vi "KYFG Scan.vi"(8 "error in (no error)":errorcluster, 10 "count":i32) -> (0 "error out":errorcluster, 2 "infosize":i32, 3 "pids_info":u32[](array[numeric]))   [LabVIEW 2023, in "KYFGLib_lv.lvlib"]
doc: "KYFG_API int KYFG_Scan(unsigned int *pids_info, int count);"
uses:
  KYFGLib_lv.lvlib
  KYFGLib.dll
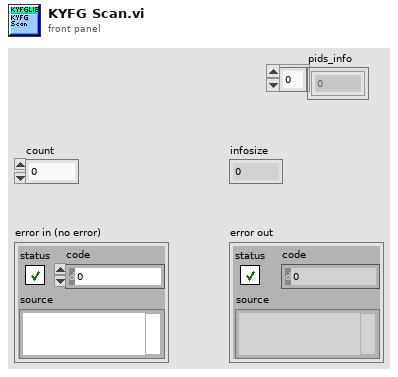
[diagram p1: front panel]
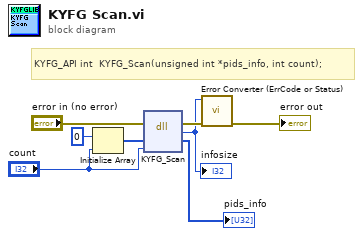
[diagram p0: block diagram]
diagram:
  # "KYFG_API int\t\tKYFG_Scan(unsigned int *pids_info, int count);"
  n1 = Initialize Array(u32 0 ("element"), "count") -> (w1:u32[])
  n2 = dll-call lib="KYFGLib.dll" fn="KYFG_Scan"(error in="error in (no error)", "pids_info"=w1, "count"="count") -> (error out=w7:errorcluster, "return type"=w5:i32, "pids_info"=→"pids_info":u32[])  [unwired: 3 in, 1 out]
  "infosize" <- w5
  n3 = call "Error Converter (ErrCode or Status).vi"("error in (no error)"=w7, "error code"=w5) -> ("error out"=→"error out":errorcluster)  [unwired: 9 in]
